vi "query(byVal).vi"(6 "use Regex? (F)":bool, 9 "Search string":string, 10 "Search Key (FQN)":T1, 11 "Instance":refnum<class "NameRegistry.lvclass">) -> (1 "Nodes":refnum<class "UniqueName.lvclass">[](array[class]), 2 "First Node":refnum<class "UniqueName.lvclass">, 3 "Instance":refnum<class "NameRegistry.lvclass">, 4 "found?":bool)   [LabVIEW 2013, in "UniqueName.lvlib" / "NameRegistry.lvclass"]
uses:
  NameRegistry.lvclass
  UniqueNameClass/UniqueName.lvclass
  <vilib>/regexp/Match Regular Expression.xnode
  UniqueNameClass/Key.ctl
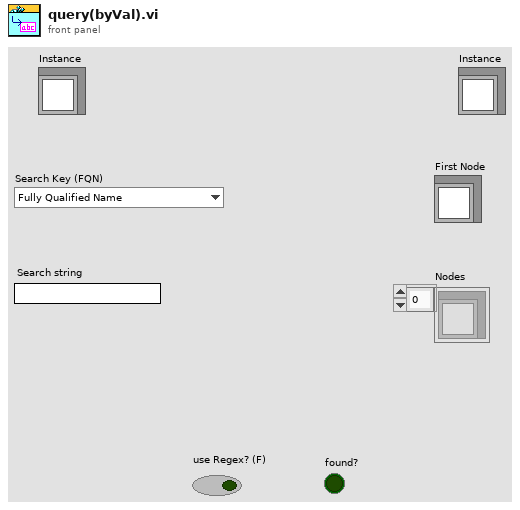
[diagram p1: front panel]
types:
  T1 = typedef "UniqueName.lvlib/UniqueName.lvclass/Key.ctl" = enum16{"Fully Qualified Name", "Unique Name", "Given Name", "Parent Fully Qualified Name", "UUID"}
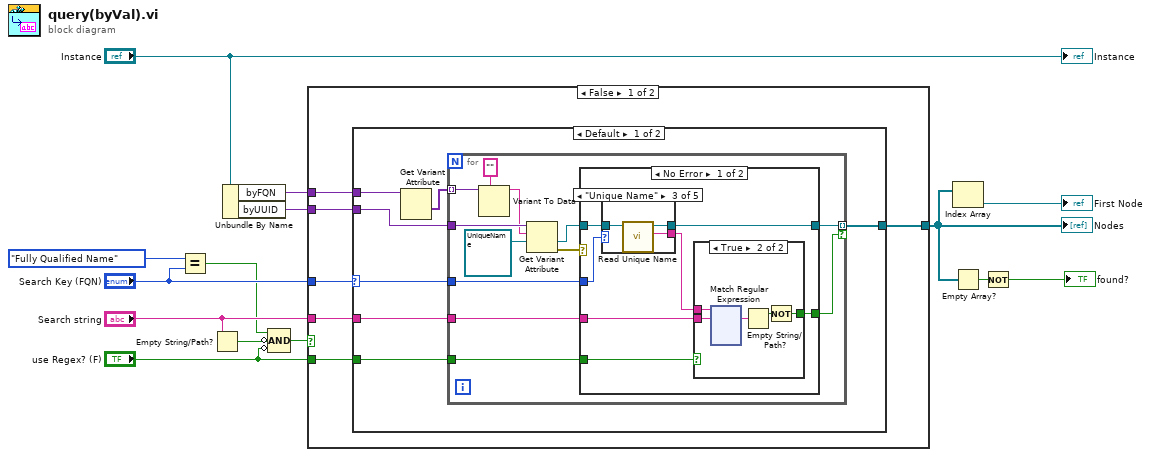
[diagram p0: block diagram]
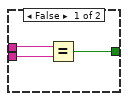
[diagram p2: hidden frame]
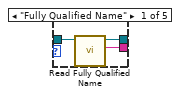
[diagram p3: hidden frame]
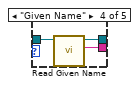
[diagram p5: hidden frame]
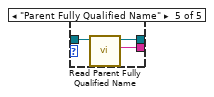
[diagram p6: hidden frame]
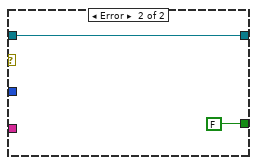
[diagram p7: hidden frame]
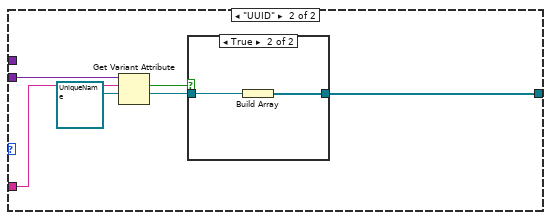
[diagram p8: hidden frame]
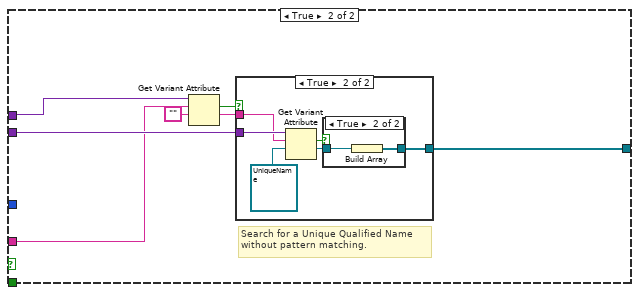
[diagram p10: hidden frame]
diagram:
  n1 = Equal?(x=Key."Fully Qualified Name", y="Search Key (FQN)") -> (x = y?=w6:bool)
  n2 = Empty String/Path?(string/path="Search string") -> (empty?=w5:bool)
  n3 = Unbundle By Name("Instance") -> ("byFQN"=w4:variant, "byUUID"=w3:variant)
  n4 = Compound Arithmetic op=AND(w6, invert w5, invert "use Regex? (F)") -> (w2:bool)
  n5 = case shown="False" w2 {
    tunnel: w3 -> [w16 w198]
    tunnel: [w20 w197] -> w10
    tunnel: "Search string" -> [w18 w195]
    tunnel: "Search Key (FQN)" -> [w15 _]
    tunnel: "use Regex? (F)" -> [w19 _]
    tunnel: w4 -> [w17 w192]
    frame False {
      n6 = case shown="Default" w15 {
        selector: w15 -> [w21 _]
        tunnel: [w27 w184] -> w20
        tunnel: w19 -> [w26 _]
        tunnel: w18 -> [w25 w188]
        tunnel: w17 -> [w24 _]
        tunnel: w16 -> [w23 w189]
        frame Default {
          n7 = Get Variant Attribute(Variant=w24) -> (values=w22:variant[])  [unwired: 3 in, 3 out]
          n8 = for {
            tunnel: w23 -> [w34]
            tunnel: [w38] -> w27 mode=indexing if=w37
            tunnel: w26 -> [w36]
            tunnel: w25 -> [w35]
            tunnel: w21 -> [w39]
            tunnel: w22 -> [w33] mode=indexing
            n9 = Variant To Data(type="", Variant=w33) -> (data=w31:string)  [unwired: 1 in, 1 out]
            n10 = Get Variant Attribute(Variant=w34, name=w31, default value (empty Variant)=refnum<class "UniqueName.lvclass"> refnum ("UniqueName.lvclass")) -> (value=w29:refnum<class "UniqueName.lvclass">, error out=w28:errorcluster)  [unwired: 1 in, 2 out]
            n11 = case shown="No Error" w28 {
              tunnel: [w40 FALSE] -> w37
              tunnel: w39 -> [w46 _]
              tunnel: w29 -> [w45 w183]
              tunnel: [w44 w183] -> w38
              tunnel: w36 -> [w43 _]
              tunnel: w35 -> [w41 _]
              frame No Error {
                n12 = case shown="\"Unique Name\"" w46 {
                  tunnel: w45 -> [w171 w172 w175 w178 w181]
                  tunnel: [w170 w172 w174 w177 w180] -> w44
                  tunnel: [w169 _ w173 w176 w179] -> w42
                  frame "Fully Qualified Name" {
                    n13 = call "Read Fully Qualified Name.vi"("UniqueName in"=w171) -> ("Fully Qualified Name"=w169:string, "UniqueName out"=w170:refnum<class "UniqueName.lvclass">)  [unwired: 9 in]
                  }
                  frame "UUID" {
                  }
                  frame "Unique Name" {
                    n14 = call "Read Unique Name.vi"("UniqueName in"=w175) -> ("Unique Name"=w173:string, "UniqueName out"=w174:refnum<class "UniqueName.lvclass">)  [unwired: 9 in]
                  }
                  frame "Given Name" {
                    n15 = call "Read Given Name.vi"("UniqueName in"=w178) -> ("Given Name"=w176:string, "UniqueName out"=w177:refnum<class "UniqueName.lvclass">)  [unwired: 9 in]
                  }
                  frame "Parent Fully Qualified Name" {
                    n16 = call "Read Parent Fully Qualified Name.vi"("UniqueName in"=w181) -> ("Parent Fully Qualified Name"=w179:string, "UniqueName out"=w180:refnum<class "UniqueName.lvclass">)  [unwired: 9 in]
                  }
                }
                n17 = case shown="True" w43 {
                  tunnel: w42 -> [w49 w54]
                  tunnel: w41 -> [w48 w53]
                  tunnel: [w47 w50] -> w40
                  frame False {
                    n18 = Equal?(x=w49, y=w48) -> (x = y?=w47:bool)
                  }
                  frame True {
                    n19 = xnode "Match Regular Expression"("input string"=w54, "regular expression"=w53) -> ("whole match"=w52:string)  [unwired: 4 in, 4 out]
                    n20 = Empty String/Path?(string/path=w52) -> (empty?=w51:bool)
                    n21 = Not(x=w51) -> (.not. x?=w50:bool)
                  }
                }
              }
              frame Error {
              }
            }
          }
        }
        frame "UUID" {
          n22 = Get Variant Attribute(Variant=w189, name=w188, default value (empty Variant)=refnum<class "UniqueName.lvclass"> refnum ("UniqueName.lvclass")) -> (found=w186:bool, value=w185:refnum<class "UniqueName.lvclass">)  [unwired: 1 in, 2 out]
          n23 = case shown="True" w186 {
            tunnel: w185 -> [_ w191]
            tunnel: [_ w190] -> w184
            frame False {
            }
            frame True {
              n24 = Build Array(w191) -> (w190:refnum<class "UniqueName.lvclass">[])
            }
          }
        }
      }
    }
    frame True {
      # "Search for a Unique Qualified Name\nwithout pattern matching."
      n25 = Get Variant Attribute(Variant=w192, name=w195, default value (empty Variant)="") -> (found=w193:bool, value=w194:string)  [unwired: 1 in, 2 out]
      n26 = case shown="True" w193 {
        tunnel: w198 -> [_ w204]
        tunnel: [_ w202] -> w197
        tunnel: w194 -> [_ w200]
        frame False {
        }
        frame True {
          n27 = Get Variant Attribute(Variant=w204, name=w200, default value (empty Variant)=refnum<class "UniqueName.lvclass"> refnum ("UniqueName Object (Set)")) -> (found=w201:bool, value=w203:refnum<class "UniqueName.lvclass">)  [unwired: 1 in, 2 out]
          n28 = case shown="True" w201 {
            tunnel: w203 -> [_ w206]
            tunnel: [_ w205] -> w202
            frame False {
            }
            frame True {
              n29 = Build Array(w206) -> (w205:refnum<class "UniqueName.lvclass">[])
            }
          }
        }
      }
    }
  }
  "Nodes" <- w10
  n30 = Index Array(array=w10) -> (element=→"First Node":refnum<class "UniqueName.lvclass">)  [unwired: 1 in]
  n31 = Empty Array?(array=w10) -> (empty?=w1:bool)
  n32 = Not(x=w1) -> (.not. x?=→"found?":bool)
  "Instance" <- "Instance"
